vi "CreateExportedFunctionVIs.vi"   [LabVIEW 2020]
uses:
  <vilib>/Utility/traverseref.llb/TRef TravTarget.ctl
  6dd5ec1a-3140-4c59-8976-e265b4825e4e.vi
  c28e3e03-bc47-4083-b8a7-f1b137712541.vi
  82b46e61-a036-43bd-a8d9-afcc1ab177d3.vi
  337b4f8b-581d-4fd9-b696-00d79b3d5e3a.vi
  67cb83f1-d3a9-42e9-95c3-879ee97d33c6.vi
  533b81a4-3358-4744-80f6-d38457af82e6.vi
  aa8324b7-c77c-40f3-a2ff-be6155b8576c.vi
  g_industrial_cam/Camera/Get Pixel Format.vi
  g_industrial_cam/Camera/Set Pixel Format.vi
  g_industrial_cam/Camera/Get Exposure Time Bounds.vi
  g_industrial_cam/Camera/Available Pixel Formats.vi
  g_industrial_cam/Camera/Is Gain Available.vi
  g_industrial_cam/Camera/Get Height Increment.vi
  g_industrial_cam/Camera/Get Gain Representation.vi
  <vilib>/Comparison/Equal/Equal Functor/Equal Functor.lvclass
  <vilib>/Utility/traverseref.llb/VI Scripting - Traverse.lvlib
  g_industrial_cam/Camera/Camera.lvclass
types:
  T1 = typedef "TRef TravTarget.ctl" = enum16{"FP", "BD", "Other"}
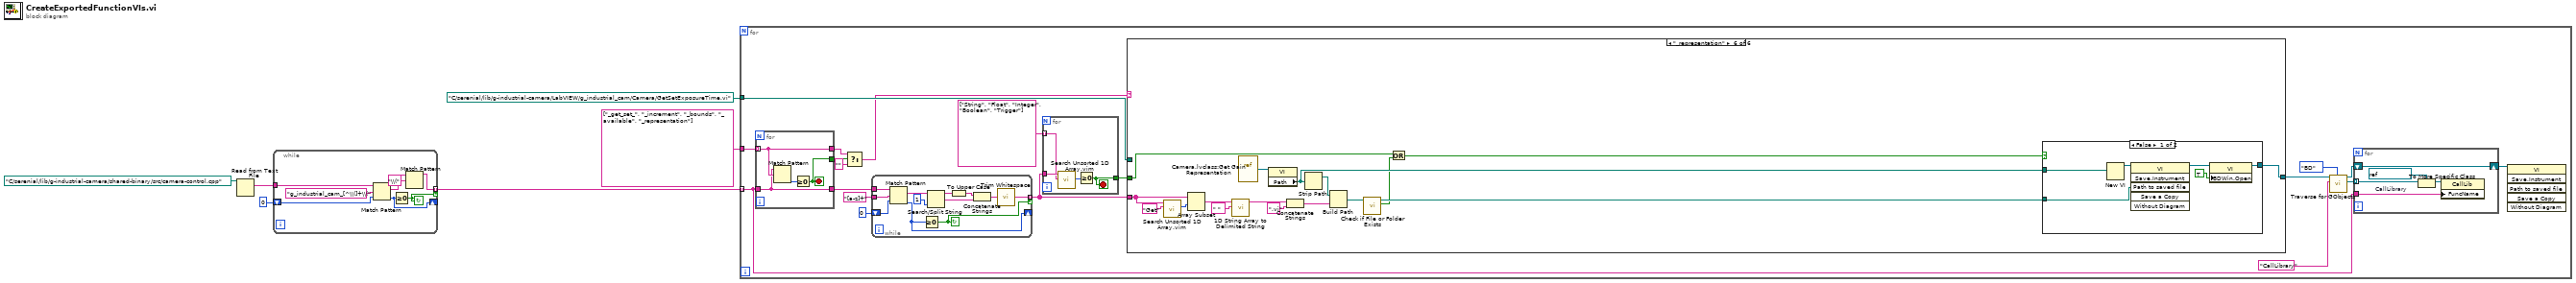
[diagram p0: block diagram]
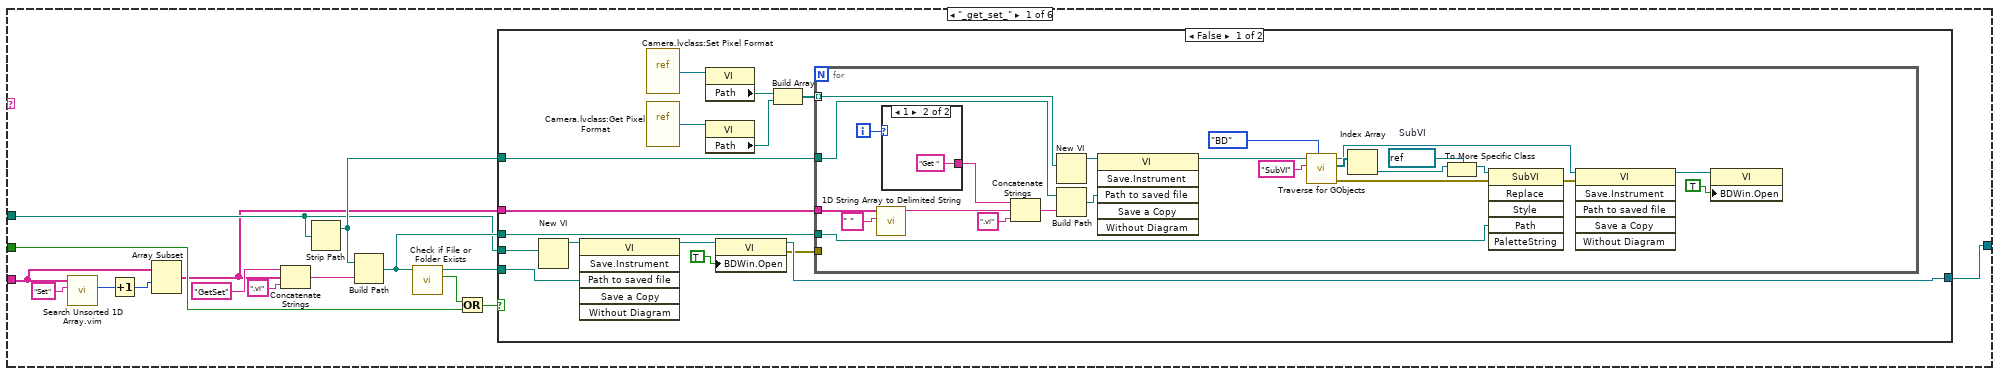
[diagram p2: hidden frame]
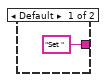
[diagram p3: hidden frame]
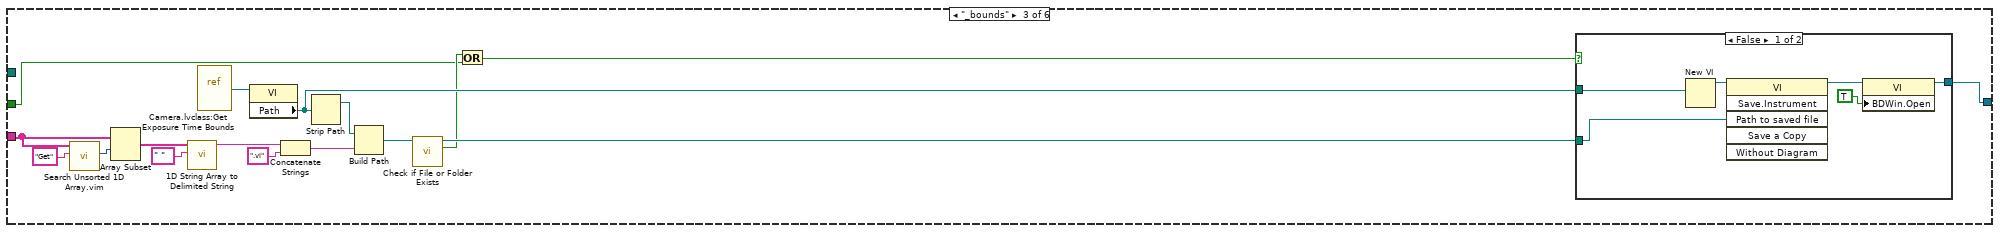
[diagram p6: hidden frame]
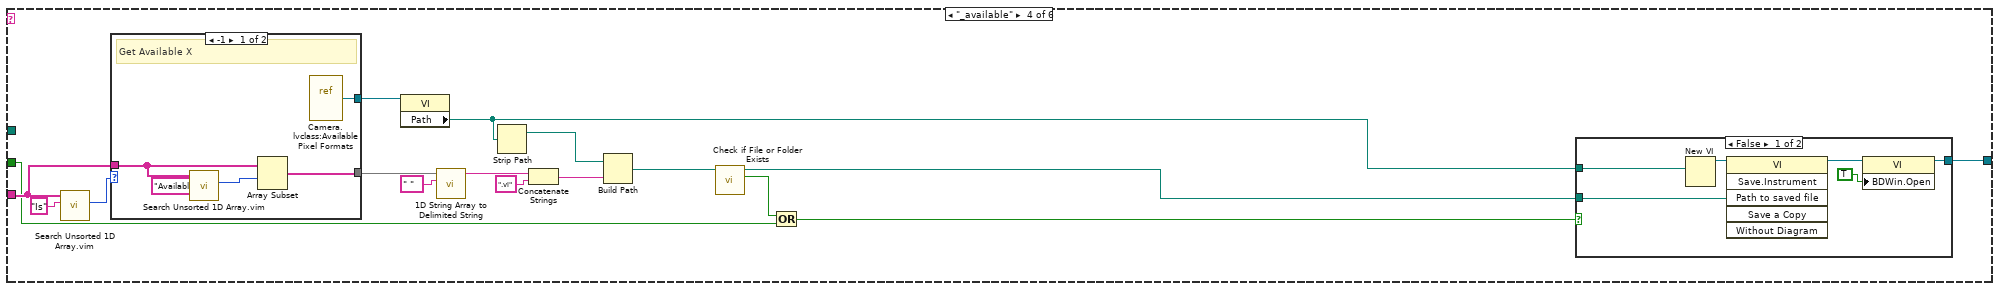
[diagram p8: hidden frame]
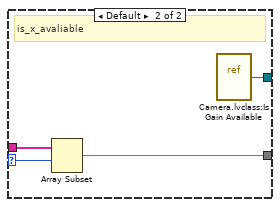
[diagram p9: hidden frame]
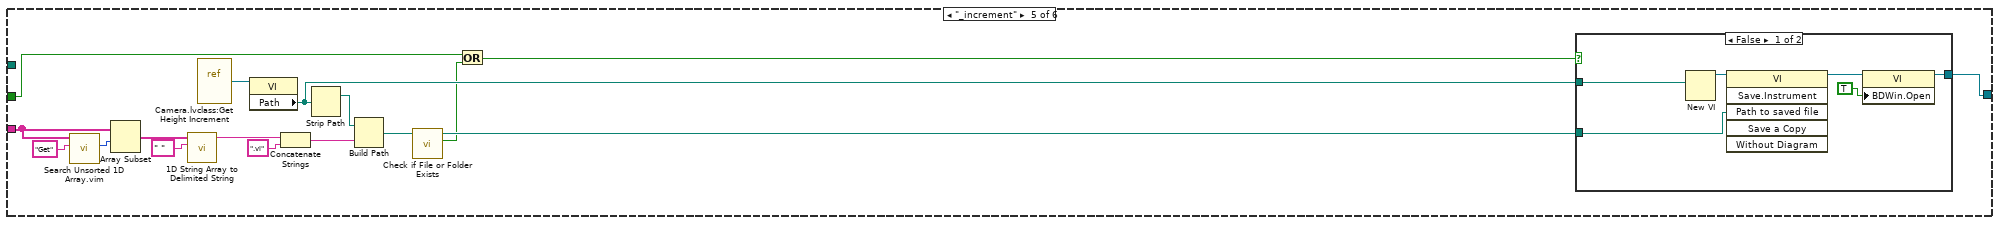
[diagram p11: hidden frame]
diagram:
  n1 = Read from Text File(file (use dialog)=path "C:/serenial/lib/g-industrial-camera/shared-binary/src/camera-control.cpp") -> (text=w1:string)  [unwired: 3 in, 3 out]
  n2 = while {
    tunnel: w1 -> [w14]
    shift-right: [w8] -> _
    shift-left: 0 ("offset (0)") -> [w12]
    tunnel: [w9] -> w5 mode=indexing if=w11
    stop <- w11 continue-if-true
    n3 = Match Pattern(string=w14, regular expression="g_industrial_cam_[^\\(]+\\(", offset (0)=w12) -> (match substring=w7:string, offset past match=w8:i32)  [unwired: 2 out]
    n4 = Greater Or Equal To 0?(x=w8) -> (x >= 0?=w11:bool)
    n5 = Match Pattern(string=w7, regular expression="\\(") -> (before substring=w9:string)  [unwired: 1 in, 3 out]
  }
  n6 = for {
    tunnel: w5 -> [w23] mode=indexing
    tunnel: string[] ["_get_set_", "_increment", "_bounds", "_available", "_representation"] -> [w33]
    tunnel: path "C:/serenial/lib/g-industrial-camera/LabVIEW/g_industrial_cam/Camera/GetSetExposureTime.vi" ("template") -> [w22]
    n7 = for {
      tunnel: w23 -> [w215]
      tunnel: w33 -> [w216] mode=indexing
      tunnel: [w216] -> w17
      tunnel: [w215] -> w32
      tunnel: [w213] -> w18
      stop <- w213 stop-if-true
      n8 = Match Pattern(string=w215, regular expression=w216) -> (offset past match=w214:i32)  [unwired: 1 in, 3 out]
      n9 = Greater Or Equal To 0?(x=w214) -> (x >= 0?=w213:bool)
    }
    n10 = Select(t=w17, s=w18, f="") -> (s? t:f=w16:string)
    n11 = while {
      tunnel: w32 -> [w54]
      tunnel: "[a-z]+" ("regular expression") -> [w53]
      shift-right: [w51] -> _
      shift-left: 0 ("offset (0)") -> [w52]
      tunnel: [w43] -> w20 mode=indexing if=w50
      stop <- w50 continue-if-true
      n12 = Match Pattern(string=w54, regular expression=w53, offset (0)=w52) -> (match substring=w48:string, offset past match=w51:i32)  [unwired: 2 out]
      n13 = Greater Or Equal To 0?(x=w51) -> (x >= 0?=w50:bool)
      n14 = Search/Split String(string=w48, offset (0)=1) -> (substring before match=w47:string, match + rest of string=w45:string)  [unwired: 1 in, 1 out]
      n15 = To Upper Case(1:w47) -> (0:w46:string)
      n16 = Concatenate Strings(w46, w45) -> (w44:string)
      n17 = call <vilib>:"Trim Whitespace.vi"("string"=w44) -> ("trimmed string"=w43:string)  [unwired: 1 in]
    }
    n18 = for {
      tunnel: string[] ["String", "Float", "Integer", "Boolean", "Trigger"] -> [w36] mode=indexing
      tunnel: w20 -> [w37]
      tunnel: [w34] -> w19
      stop <- w34 stop-if-true
      n19 = call "Search Unsorted 1D Array.vim"("element"=w36, "unsorted 1D array"=w37) -> ("index of element"=w35:i32)  [unwired: 9 in]
      n20 = Greater Or Equal To 0?(x=w35) -> (x >= 0?=w34:bool)
    }
    n21 = case shown="\"_representation\"" w16 {
      tunnel: w20 -> [w62 _ w127 w150 w182 w205]
      tunnel: [w68 _ w116 w139 w171 w194] -> w26
      tunnel: w22 -> [w60 _ _ _ _ _]
      tunnel: w19 -> [w56 _ w112 w135 w167 w191]
      frame "_get_set_" {
        n22 = call "Search Unsorted 1D Array.vim"("element"="Set", "unsorted 1D array"=w62) -> ("index of element"=w63:i32)  [unwired: 9 in]
        n23 = Increment(x=w63) -> (x+1=w61:i32)
        n24 = Array Subset(array=w62, index=w61) -> (w55:string[])  [unwired: 1 in]
        n25 = Concatenate Strings("GetSet" ("string"), w55, ".vi" ("string")) -> (w69:string)
        n26 = Strip Path(path=w60) -> (stripped path=w67:path)  [unwired: 1 out]
        n27 = Build Path(base path=w67, name or relative path=w69) -> (appended path=w66:path)
        n28 = call <vilib>:"Check if File or Folder Exists.vi"("path"=w66) -> ("file or folder exists?"=w58:bool, "dup path"=w59:path)  [unwired: 8 in, 1 out]
        n29 = Or(x=w58, y=w56) -> (x .or. y?=w57:bool)
        n30 = case shown="False" w57 {
          tunnel: [w85 _] -> w68
          tunnel: w67 -> [w79 _]
          tunnel: w66 -> [w78 _]
          tunnel: w55 -> [w73 _]
          tunnel: w60 -> [w72 _]
          tunnel: w59 -> [w71 _]
          frame False {
            n31 = New VI(10:w72) -> (3:w76:refnum<vi>)  [unwired: 6 in, 1 out]
            n32 = invoke class="VI" method="Save.Instrument"(reference=w76, "Path to saved file"=w71) -> (reference out=w75:refnum<vi>)  [unwired: 4 in, 5 out]
            n33 = vi-ref "Camera.lvclass:Set Pixel Format.vi"() -> (w83:refnum<vi>)
            n34 = vi-ref "Camera.lvclass:Get Pixel Format.vi"() -> (w84:refnum<vi>)
            n35 = property class="VI"(reference=w83) -> ("Path"=w81:path)  [unwired: 1 in, 2 out]
            n36 = property class="VI"(reference=w84) -> ("Path"=w82:path)  [unwired: 1 in, 2 out]
            n37 = property class="VI"(reference=w75, "BDWin.Open"=TRUE ("Block Diagram Window:Open")) -> (reference out=w85:refnum<vi>, error out=w77:errorcluster)  [unwired: 1 in]
            n38 = Build Array(w81, w82) -> (w80:path[])
            n39 = for {
              tunnel: w80 -> [w104] mode=indexing
              tunnel: w79 -> [w105]
              tunnel: w73 -> [w102]
              tunnel: w78 -> [w103]
              tunnel: w77 -> [_]
              i -> [w101]
              w92 = refnum<vi> refnum  # SubVI
              n40 = call <vilib>:"1D String Array to Delimited String.vi"("delimiter"=" ", "string array"=w102) -> ("delimited string"=w108:string)  [unwired: 9 in]
              n41 = case shown="1" w101 {
                tunnel: ["Set " "Get "] -> w100
                frame Default {
                }
                frame 1 {
                }
              }
              n42 = Concatenate Strings(w100, w108, ".vi" ("string")) -> (w106:string)
              n43 = New VI(10:w104) -> (3:w99:refnum<vi>)  [unwired: 6 in, 1 out]
              n44 = Build Path(base path=w105, name or relative path=w106) -> (appended path=w98:path)
              n45 = invoke class="VI" method="Save.Instrument"(reference=w99, "Path to saved file"=w98) -> (reference out=w97:refnum<vi>)  [unwired: 4 in, 5 out]
              n46 = call <vilib>:"Traverse for GObjects.vi"("Traverse Target"=TRef_TravTarget."BD", "Class Name"="SubVI", "VI Refnum"=w97) -> ("error out"=w90:errorcluster, "References"=w94:refnum<vi>[], "dup VI Refnum"=w89:refnum<vi>)  [unwired: 5 in, 1 out]
              n47 = Index Array(array=w94) -> (element=w93:refnum<vi>)  [unwired: 1 in]
              n48 = To More Specific Class(target class=w92, reference=w93) -> (specific class reference=w91:refnum<vi>)  [unwired: 1 in, 1 out]
              n49 = invoke class="SubVI" method="Replace"(reference=w91, error in=w90, "Path"=w103) -> (error out=w88:errorcluster)  [unwired: 3 in, 5 out]
              n50 = invoke class="VI" method="Save.Instrument"(reference=w89, error in=w88) -> (reference out=w87:refnum<vi>)  [unwired: 4 in, 5 out]
              n51 = property class="VI"(reference=w87, "BDWin.Open"=TRUE ("Block Diagram Window:Open")) -> ()  [unwired: 1 in, 2 out]
            }
          }
          frame True {
          }
        }
      }
      frame Default {
      }
      frame "_bounds" {
        n52 = call "Search Unsorted 1D Array.vim"("element"="Get", "unsorted 1D array"=w127) -> ("index of element"=w126:i32)  [unwired: 9 in]
        n53 = Array Subset(array=w127, index=w126) -> (w123:string[])  [unwired: 1 in]
        n54 = call <vilib>:"1D String Array to Delimited String.vi"("delimiter"=" ", "string array"=w123) -> ("delimited string"=w121:string)  [unwired: 9 in]
        n55 = vi-ref "Camera.lvclass:Get Exposure Time Bounds.vi"() -> (w125:refnum<vi>)
        n56 = property class="VI"(reference=w125) -> ("Path"=w120:path)  [unwired: 1 in, 2 out]
        n57 = Concatenate Strings(w121, ".vi" ("string")) -> (w118:string)
        n58 = Strip Path(path=w120) -> (stripped path=w119:path)  [unwired: 1 out]
        n59 = Build Path(base path=w119, name or relative path=w118) -> (appended path=w117:path)
        n60 = call <vilib>:"Check if File or Folder Exists.vi"("path"=w117) -> ("file or folder exists?"=w114:bool, "dup path"=w115:path)  [unwired: 8 in, 1 out]
        n61 = Or(x=w114, y=w112) -> (x .or. y?=w113:bool)
        n62 = case shown="False" w113 {
          tunnel: w120 -> [w133 _]
          tunnel: [w130 _] -> w116
          tunnel: w115 -> [w129 _]
          frame False {
            n63 = New VI(10:w133) -> (3:w134:refnum<vi>)  [unwired: 6 in, 1 out]
            n64 = invoke class="VI" method="Save.Instrument"(reference=w134, "Path to saved file"=w129) -> (reference out=w132:refnum<vi>)  [unwired: 4 in, 5 out]
            n65 = property class="VI"(reference=w132, "BDWin.Open"=TRUE ("Block Diagram Window:Open")) -> (reference out=w130:refnum<vi>)  [unwired: 1 in, 1 out]
          }
          frame True {
          }
        }
      }
      frame "_available" {
        n66 = call "Search Unsorted 1D Array.vim"("element"="Is", "unsorted 1D array"=w150) -> ("index of element"=w149:i32)  [unwired: 9 in]
        n67 = case shown="-1" w149 {
          selector: w149 -> [_ w159]
          tunnel: w150 -> [w155 w160]
          tunnel: [w152 w158] -> w148
          tunnel: [w153 w157] -> w146
          frame -1 {
            # "Get Available X"
            n68 = call "Search Unsorted 1D Array.vim"("element"="Available", "unsorted 1D array"=w155) -> ("index of element"=w154:i32)  [unwired: 9 in]
            n69 = Array Subset(array=w155, index=w154) -> (w153:string[])  [unwired: 1 in]
            n70 = vi-ref "Camera.lvclass:Available Pixel Formats.vi"() -> (w152:refnum<vi>)
          }
          frame Default {
            # "is_x_avaliable"
            n71 = Array Subset(array=w160, index=w159) -> (w157:string[])  [unwired: 1 in]
            n72 = vi-ref "Camera.lvclass:Is Gain Available.vi"() -> (w158:refnum<vi>)
          }
        }
        n73 = property class="VI"(reference=w148) -> ("Path"=w143:path)  [unwired: 1 in, 2 out]
        n74 = call <vilib>:"1D String Array to Delimited String.vi"("delimiter"=" ", "string array"=w146) -> ("delimited string"=w144:string)  [unwired: 9 in]
        n75 = Strip Path(path=w143) -> (stripped path=w142:path)  [unwired: 1 out]
        n76 = Concatenate Strings(w144, ".vi" ("string")) -> (w141:string)
        n77 = Build Path(base path=w142, name or relative path=w141) -> (appended path=w140:path)
        n78 = call <vilib>:"Check if File or Folder Exists.vi"("path"=w140) -> ("file or folder exists?"=w137:bool, "dup path"=w138:path)  [unwired: 8 in, 1 out]
        n79 = Or(x=w137, y=w135) -> (x .or. y?=w136:bool)
        n80 = case shown="False" w136 {
          tunnel: w143 -> [w165 _]
          tunnel: [w162 _] -> w139
          tunnel: w138 -> [w161 _]
          frame False {
            n81 = New VI(10:w165) -> (3:w166:refnum<vi>)  [unwired: 6 in, 1 out]
            n82 = invoke class="VI" method="Save.Instrument"(reference=w166, "Path to saved file"=w161) -> (reference out=w164:refnum<vi>)  [unwired: 4 in, 5 out]
            n83 = property class="VI"(reference=w164, "BDWin.Open"=TRUE ("Block Diagram Window:Open")) -> (reference out=w162:refnum<vi>)  [unwired: 1 in, 1 out]
          }
          frame True {
          }
        }
      }
      frame "_increment" {
        n84 = call "Search Unsorted 1D Array.vim"("element"="Get", "unsorted 1D array"=w182) -> ("index of element"=w181:i32)  [unwired: 9 in]
        n85 = Array Subset(array=w182, index=w181) -> (w178:string[])  [unwired: 1 in]
        n86 = call <vilib>:"1D String Array to Delimited String.vi"("delimiter"=" ", "string array"=w178) -> ("delimited string"=w176:string)  [unwired: 9 in]
        n87 = vi-ref "Camera.lvclass:Get Height Increment.vi"() -> (w180:refnum<vi>)
        n88 = property class="VI"(reference=w180) -> ("Path"=w175:path)  [unwired: 1 in, 2 out]
        n89 = Concatenate Strings(w176, ".vi" ("string")) -> (w173:string)
        n90 = Strip Path(path=w175) -> (stripped path=w174:path)  [unwired: 1 out]
        n91 = Build Path(base path=w174, name or relative path=w173) -> (appended path=w172:path)
        n92 = call <vilib>:"Check if File or Folder Exists.vi"("path"=w172) -> ("file or folder exists?"=w169:bool, "dup path"=w170:path)  [unwired: 8 in, 1 out]
        n93 = Or(x=w167, y=w169) -> (x .or. y?=w168:bool)
        n94 = case shown="False" w168 {
          tunnel: w175 -> [w188 _]
          tunnel: [w185 _] -> w171
          tunnel: w170 -> [w184 _]
          frame False {
            n95 = New VI(10:w188) -> (3:w189:refnum<vi>)  [unwired: 6 in, 1 out]
            n96 = invoke class="VI" method="Save.Instrument"(reference=w189, "Path to saved file"=w184) -> (reference out=w187:refnum<vi>)  [unwired: 4 in, 5 out]
            n97 = property class="VI"(reference=w187, "BDWin.Open"=TRUE ("Block Diagram Window:Open")) -> (reference out=w185:refnum<vi>)  [unwired: 1 in, 1 out]
          }
          frame True {
          }
        }
      }
      frame "_representation" {
        n98 = call "Search Unsorted 1D Array.vim"("element"="Get", "unsorted 1D array"=w205) -> ("index of element"=w204:i32)  [unwired: 9 in]
        n99 = Array Subset(array=w205, index=w204) -> (w201:string[])  [unwired: 1 in]
        n100 = call <vilib>:"1D String Array to Delimited String.vi"("delimiter"=" ", "string array"=w201) -> ("delimited string"=w199:string)  [unwired: 9 in]
        n101 = vi-ref "Camera.lvclass:Get Gain Representation.vi"() -> (w203:refnum<vi>)
        n102 = property class="VI"(reference=w203) -> ("Path"=w198:path)  [unwired: 1 in, 2 out]
        n103 = Concatenate Strings(w199, ".vi" ("string")) -> (w196:string)
        n104 = Strip Path(path=w198) -> (stripped path=w197:path)  [unwired: 1 out]
        n105 = Build Path(base path=w197, name or relative path=w196) -> (appended path=w195:path)
        n106 = call <vilib>:"Check if File or Folder Exists.vi"("path"=w195) -> ("file or folder exists?"=w192:bool, "dup path"=w193:path)  [unwired: 8 in, 1 out]
        n107 = Or(x=w191, y=w192) -> (x .or. y?=w190:bool)
        n108 = case shown="False" w190 {
          tunnel: w198 -> [w211 _]
          tunnel: [w208 _] -> w194
          tunnel: w193 -> [w207 _]
          frame False {
            n109 = New VI(10:w211) -> (3:w212:refnum<vi>)  [unwired: 6 in, 1 out]
            n110 = invoke class="VI" method="Save.Instrument"(reference=w212, "Path to saved file"=w207) -> (reference out=w210:refnum<vi>)  [unwired: 4 in, 5 out]
            n111 = property class="VI"(reference=w210, "BDWin.Open"=TRUE ("Block Diagram Window:Open")) -> (reference out=w208:refnum<vi>)  [unwired: 1 in, 1 out]
          }
          frame True {
          }
        }
      }
    }
    n112 = call <vilib>:"Traverse for GObjects.vi"("Traverse Target"=TRef_TravTarget."BD", "Class Name"="CallLibrary", "VI Refnum"=w26) -> ("References"=w27:refnum<vi>[], "dup VI Refnum"=w25:refnum<vi>)  [unwired: 5 in, 2 out]
    n113 = for {
      tunnel: w27 -> [w41] mode=indexing
      tunnel: w23 -> [w39]
      shift-right: [w38] -> w24
      shift-left: w25 -> [w38]
      w42 = refnum<vi> refnum  # CallLibrary
      n114 = To More Specific Class(target class=w42, reference=w41) -> (specific class reference=w40:refnum<vi>)  [unwired: 1 in, 1 out]
      n115 = property class="CallLib"(reference=w40, "FuncName"=w39) -> ()  [unwired: 1 in, 2 out]
    }
    n116 = invoke class="VI" method="Save.Instrument"(reference=w24) -> ()  [unwired: 5 in, 6 out]
  }
